vi "Copy python module.vi"(11 "Test Case In":refnum<class "Runner Unit Test - Prepare Project.lvclass">) -> (0 "error out":errorcluster, 3 "Test Case Out":refnum<class "Runner Unit Test - Prepare Project.lvclass">)   [LabVIEW 2026, in "Runner Unit Test - Prepare Project.lvclass"]
uses:
  Runner Unit Test - Prepare Project.lvclass
  C:/Program Files/National Instruments/LabVIEW 2026/vi.lib/Astemes/LUnit/Test Case.lvclass
  Actors/Runner/Runner/Runner.lvclass
  Interfaces/IRunner/IRunner/Interfaces--cluster.ctl
  Interfaces/IProject Manager/IProject Manager.lvclass
  Interfaces/IFile Manager/IFile Manager.lvclass
  Interfaces/IPython Caller/IPython Caller.lvclass
  Interfaces/IElement Manager/IElement Manager.lvclass
  Interfaces/ILV File Creator/ILV File Creator.lvclass
  Interfaces/IHash Whitelist Handler/IHash Whitelist Handler.lvclass
  Actors/Mock Logger/Mock Logger/Mock Logger.lvclass
  C:/Program Files/National Instruments/LabVIEW 2026/vi.lib/ActorFramework/Actor/Actor.lvclass
  <vilib>/ActorFramework/Message Enqueuer/Message Enqueuer.lvclass/Message Enqueuer.ctl
  <vilib>/ActorFramework/Message Enqueuer/Enqueue.vi
  Mocks/Mock IFile Manager/Mock IFile Manager.lvclass
  C:/Program Files/National Instruments/LabVIEW 2026/vi.lib/Astemes/LMock/Mock.lvclass
  C:/Users/juanj/Documents/hasbun_wood_engineering/github/py2vi/labview/Interfaces/IFile Manager/IFile Manager.lvclass
  <vilib>/ActorFramework/Stop Msg/Stop Msg.lvclass
  C:/Program Files/National Instruments/LabVIEW 2026/vi.lib/ActorFramework/Message/Message.lvclass
  <vilib>/Astemes/LMock/One Identical Inputs.vi
  <vilib>/ActorFramework/Message Priority Queue/Priority Enqueue.vi
  Runner Unit Test - Prepare Project.lvclass/Runner Unit Test - Prepare Project.ctl
  C:/Users/juanj/Documents/hasbun_wood_engineering/github/py2vi/labview/Mocks/Mock IFile Manager/Mock IFile Manager.lvclass
  Interfaces/IRunner/IRunner/IRunner.lvclass
  <vilib>/ActorFramework/Actor/Actor.lvclass
  <vilib>/Astemes/LMock/LMock Verifier.lvclass
  <vilib>/Astemes/LMock/LMock.lvlib
  <vilib>/Astemes/LMock/LMock One.lvlib
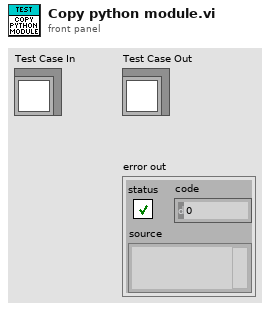
[diagram p1: front panel]
types:
  T1 = typedef "IRunner.lvlib/IRunner.lvclass/Interfaces--cluster.ctl" = cluster{"IProject Manager":refnum<class "IProject Manager.lvclass">, "IFile Manager":refnum<class "IFile Manager.lvclass">, "IPython Caller":refnum<class "IPython Caller.lvclass">, "IElement Manager":refnum<class "IElement Manager.lvclass">, "ILV File Creator":refnum<class "ILV File Creator.lvclass">, "IHash Whitelist Handler":refnum<class "IHash Whitelist Handler.lvclass">}
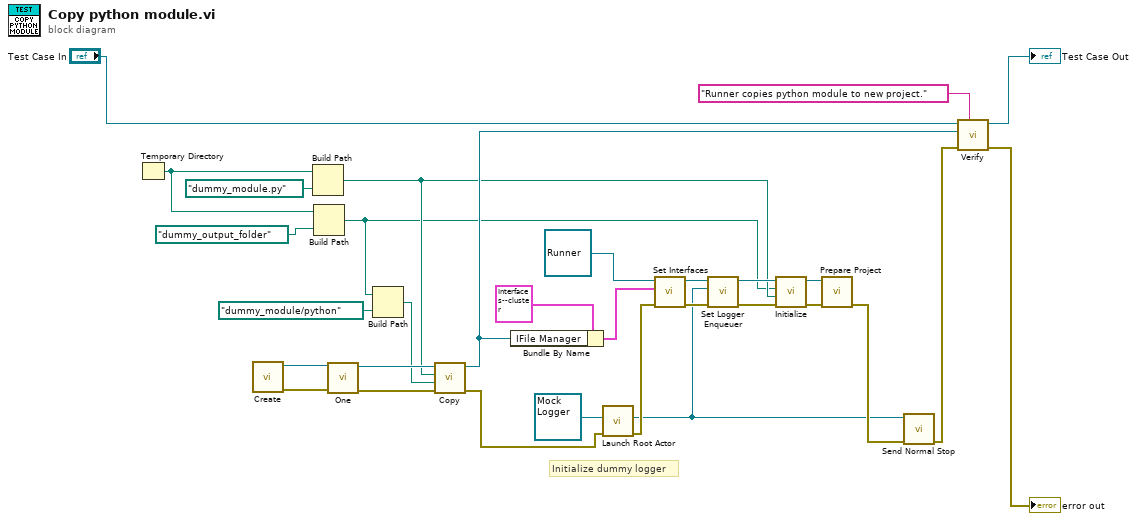
[diagram p0: block diagram]
diagram:
  # "Initialize dummy logger"
  n1 = Temporary Directory() -> (w9:path)
  n2 = call "Create.vi"() -> ("error out"=w30:errorcluster, "Mock Class Generator out"=w17:refnum<class "Mock IFile Manager.lvclass">)  [unwired: 10 in]
  n3 = Build Path(base path=w9, name or relative path=path "dummy_module.py") -> (appended path=w4:path)
  n4 = Build Path(base path=w9, name or relative path=path "dummy_output_folder") -> (appended path=w2:path)
  n5 = call-poly <vilib>:"One.vi"("error in (no error)"=w30, "Mock in"=w17) -> ("error out"=w29:errorcluster, "Mock out"=w16:refnum<class "Mock IFile Manager.lvclass">)  [unwired: 8 in]
  n6 = Build Path(base path=w2, name or relative path=path "dummy_module/python") -> (appended path=w1:path)
  n7 = call-dynamic "Copy.vi"("error in"=w29, "Target Folder"=w1, "Source File"=w4, "IFile Manager in"=w16) -> ("error out"=w23:errorcluster, "IFile Manager out"=w15:refnum<class "Mock IFile Manager.lvclass">)  [unwired: 5 in, 1 out]
  n8 = Bundle By Name(cluster=T1 {"IProject Manager"=refnum, "IFile Manager"=refnum, "IPython Caller"=refnum, "IElement Manager"=refnum, "ILV File Creator"=refnum, "IHash Whitelist Handler"=refnum} ("Interfaces"), "IFile Manager"=w15) -> (w18:T1)
  n9 = call <vilib>:"Launch Root Actor.vi"("error in (no error)"=w23, "Actor"=refnum<class "Mock Logger.lvclass"> refnum ("Mock Logger.lvlib:Mock Logger.lvclass")) -> ("error out"=w28:errorcluster, "Actor's Enqueuer"=w13:refnum<class "Message Enqueuer.lvclass">)  [unwired: 8 in]
  n10 = call-dynamic "Set Interfaces.vi"("error in"=w28, "Interfaces"=w18, "Runner in"=refnum<class "Runner.lvclass"> refnum ("Runner.lvlib:Runner.lvclass")) -> ("error out"=w31:errorcluster, "Runner out"=w20:refnum<class "Runner.lvclass">)  [unwired: 7 in]
  n11 = call-dynamic "Set Logger Enqueuer.vi"("error in"=w31, "Logger"=w13, "Runner in"=w20) -> ("error out"=w25:errorcluster, "Runner out"=w11:refnum<class "Runner.lvclass">)  [unwired: 7 in]
  n12 = call-dynamic "Initialize.vi"("error in"=w25, "Python Module"=w4, "Output Folder"=w2, "G-CLI Runner in"=w11) -> ("error out"=w24:errorcluster, "G-CLI Runner out"=w10:refnum<class "Runner.lvclass">)  [unwired: 6 in]
  n13 = call-dynamic "Prepare Project.vi"("error in"=w24, "G-CLI Runner in"=w10) -> ("error out"=w27:errorcluster)  [unwired: 8 in, 1 out]
  n14 = call <vilib>:"Send Normal Stop.vi"("error in (no error)"=w27, "Message Enqueuer"=w13) -> ("error out"=w26:errorcluster)  [unwired: 9 in]
  n15 = call <vilib>:"Verify.vi"("Description"="Runner copies python module to new project.", "error in (no error)"=w26, "Mock"=w15, "LUnit Test Case In"="Test Case In") -> ("error out"=→"error out":errorcluster, "LUnit Test Case Out"=→"Test Case Out":refnum<class "Runner Unit Test - Prepare Project.lvclass">)  [unwired: 6 in]
